vi "libssh2_agent_userauth.vi"(8 "error in (no error)":errorcluster, 9 "public key":T1, 10 "username":string, 11 "agent":T2) -> (0 "error out":errorcluster, 2 "authenticated":bool)   [LabVIEW 2017, in "libssh2.lvlib"]
doc: "Authenticate a session with a public key from an SSH agent."
uses:
  libssh2.lvlib
  Agent Refnum.ctl
  Agent Public Key Refnum.ctl
  Acquire Session.vi
  Release Session.vi
  Not An Agent.vi
  <vilib>/Utility/error.llb/Error Cluster From Error Code.vi
  Not An Agent Public Key.vi
  Global Settings.vi
  Read Agent Refnum.vi
  Read Session Refnum.vi
  <vilib>/Utility/semaphor.llb/Acquire Semaphore.vi
  <vilib>/Utility/semaphor.llb/Release Semaphore.vi
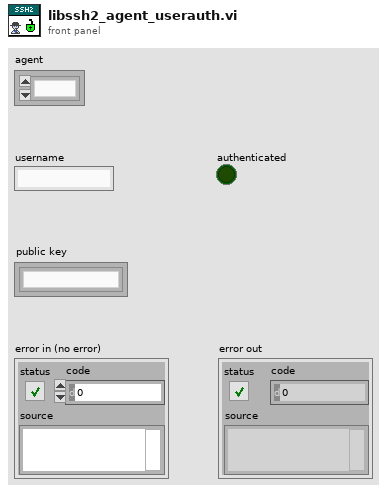
[diagram p1: front panel]
types:
  T1 = typedef "libssh2.lvlib/Agent Public Key Refnum.ctl" = refnum<k1>
  T2 = typedef "libssh2.lvlib/Agent Refnum.ctl" = refnum<k1>
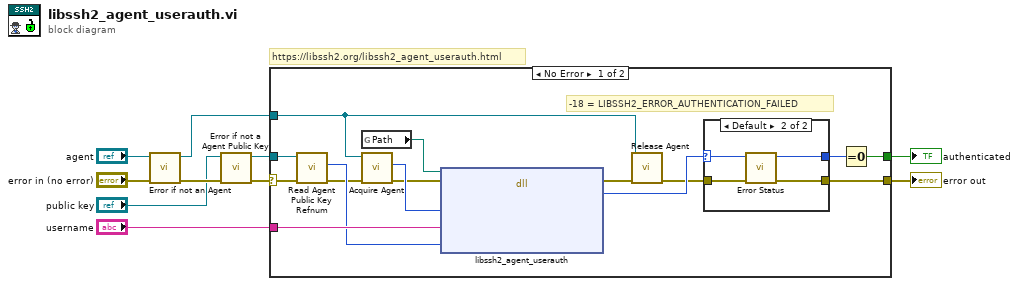
[diagram p0: block diagram]
diagram:
  # "https://libssh2.org/libssh2_agent_userauth.html"
  n1 = call "Error if not an Agent.vi"("error in (no error)"="error in (no error)", "agent"="agent") -> ("error out"=w6:errorcluster, "agent out"=w4:T2)  [unwired: 8 in]
  n2 = call "Error if not a Agent Public Key.vi"("error in (no error)"=w6, "agent public key"="public key") -> ("error out"=w3:errorcluster, "agent public key out"=w1:T1)  [unwired: 8 in]
  n3 = case shown="No Error" w3 {
    selector: w3 -> [w14 w32]
    tunnel: [w25 w32] -> w10
    tunnel: w1 -> [w23 _]
    tunnel: "username" -> [w24 _]
    tunnel: [w22 _] -> w7
    tunnel: w4 -> [w11 _]
    frame No Error {
      # "-18 = LIBSSH2_ERROR_AUTHENTICATION_FAILED"
      n4 = call "Read Agent Public Key Refnum.vi"("error in (no error)"=w14, "agent public key"=w23) -> ("error out"=w13:errorcluster, "libssh2_agent_publickey*"=w18:u64)  [unwired: 7 in, 1 out]
      n5 = global read "Global Settings.vi" "Path"() -> (w21:path)
      n6 = call "Acquire Agent.vi"("error in (no error)"=w13, "agent"=w11) -> ("error out"=w15:errorcluster, "LIBSSH2_AGENT*"=w20:u64)  [unwired: 8 in]
      n7 = dll-call lib="?" fn="libssh2_agent_userauth"(path in=w21, error in=w15, "agent"=w20, "username"=w24, "identity"=w18) -> (error out=w19:errorcluster, "return value"=w17:i32)  [unwired: 4 in, 1 out]
      n8 = call "Release Agent.vi"("error in (no error)"=w19, "agent"=w11) -> ("error out"=w12:errorcluster)  [unwired: 9 in]
      n9 = case shown="Default" w17 {
        selector: w17 -> [w26 w29]
        tunnel: w12 -> [w27 w31]
        tunnel: [w27 w30] -> w25
        tunnel: [w26 w28] -> w16
        frame -18 {
        }
        frame Default {
          n10 = call "Error Status.vi"("error in (no error)"=w31, "return value"=w29) -> ("error out"=w30:errorcluster, "return value out"=w28:i32)  [unwired: 8 in]
        }
      }
      n11 = Equal To 0?(x=w16) -> (x = 0?=w22:bool)
    }
    frame Error {
    }
  }
  "error out" <- w10
  "authenticated" <- w7
